vi "Purge uService from local lists.vi"(10 "Last Ack":refnum<class "Last Ack.lvclass">, 11 "Guardian in":refnum<class "Guardian.lvclass">) -> (0 "error out":errorcluster, 1 "uService ID":string, 2 "uService Properties":T1, 3 "Guardian out":refnum<class "Guardian.lvclass">)   [LabVIEW 2020, in "TALOS.lvlib" / "Guardian.lvlib" / "Guardian.lvclass"]
uses:
  Guardian.lvclass
  Guardian.lvclass/Guardian.ctl
  Classes/uService List/uService List.lvclass
  builds/Actor Framework PPL/Actor Framework.lvlibp/1abvi3w/vi.lib/ActorFramework/Message Enqueuer/Message Enqueuer.lvclass
  Classes/uService List/uService Properties.ctl
  TALOS.lvlib
  builds/Actor Framework PPL/Actor Framework.lvlibp/1abvi3w/vi.lib/ActorFramework/LastAck/Last Ack.lvclass
  C:/LabVIEW Code/TALOS/talos/Ancestor/Ancestor/Ancestor.lvclass
  C:/LabVIEW Code/TALOS/builds/Actor Framework PPL/Actor Framework.lvlibp/1abvi3w/vi.lib/ActorFramework/Actor/Actor.lvclass
  C:/LabVIEW Code/TALOS/talos/Guardian/Guardian/Guardian.lvclass
  Classes/Distributed uService Map/Distributed uService Map.lvclass
  Classes/uService List/Get ID from Queue.vi
  Classes/uService List/Remove uService.vi
  Classes/uService List/Get Properties.vi
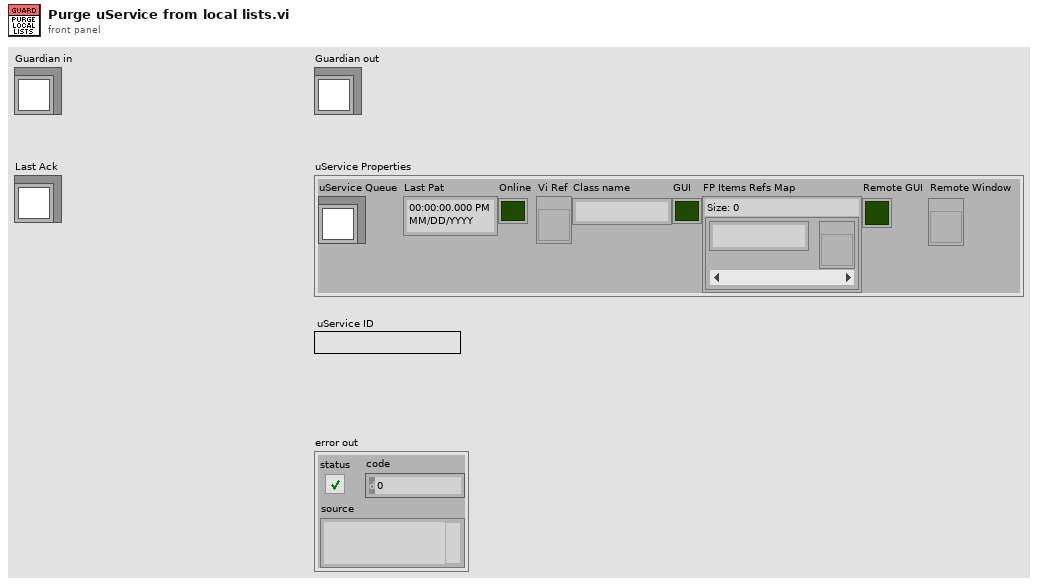
[diagram p1: front panel]
types:
  T1 = typedef "TALOS.lvlib/Classes.lvlib/uService List.lvclass/uService Properties.ctl" = cluster{"uService Queue":refnum<class "Message Enqueuer.lvclass">, "Last Pat":timestamp, "Online":bool, "Vi Ref":refnum<vi>, "Class name":string, "GUI":bool, "FP Items Refs Map":map{string, refnum<vi>}, "Remote GUI":bool, "Remote Window":refnum<vi>}
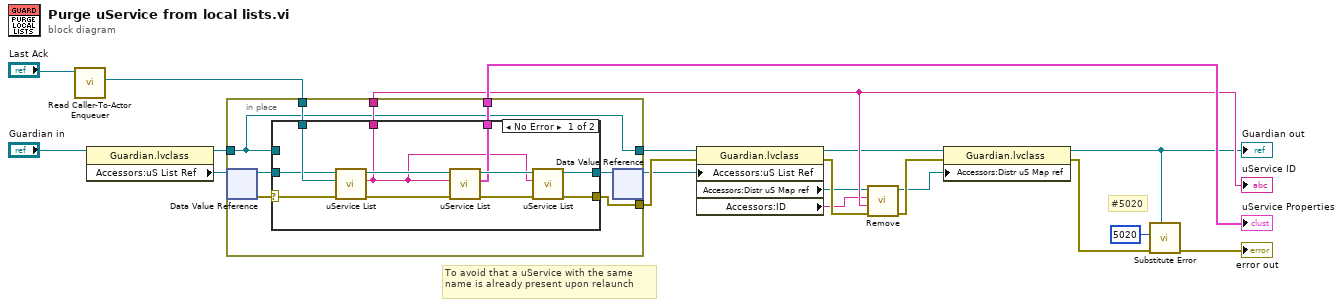
[diagram p0: block diagram]
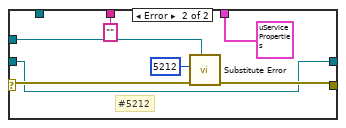
[diagram p2: hidden frame]
diagram:
  # "#5020"
  # "To avoid that a uService with the same name is already present upon relaunch"
  n1 = call "Read Caller-To-Actor Enqueuer.vi"("Last Ack"="Last Ack") -> ("Caller-to-Actor Enqueuer"=w12:refnum<class "Message Enqueuer.lvclass">)  [unwired: 10 in]
  n2 = property class="Guardian.lvclass"(reference="Guardian in") -> (reference out=w16:refnum<class "Guardian.lvclass">, "Accessors:uS List Ref"=w11:refnum<data-value>)  [unwired: 1 in, 1 out]
  n3 = in-place {
    in-place-border: w12 -> [w28]
    in-place-border: [w23] -> w18
    in-place-border: [w26] -> w14
    in-place-border: [w25] -> w19
    in-place-border: w16 -> [w21]
    in-place-border: [w21] -> w17
    n4 = in-place-dvr #1(w11) -> (w27:refnum<class "uService List.lvclass">, w22:errorcluster)
    n5 = case shown="No Error" w22 {
      selector: w22 -> [w29 w45]
      tunnel: w28 -> [w35 _]
      tunnel: w27 -> [w34 w40]
      tunnel: [w33 w43] -> w26
      tunnel: [w32 T1 {"uService Queue"=refnum, "Last Pat"=timestamp(0 s since 1904-01-01), "Online"=FALSE, "Vi Ref"=refnum, "Class name"="", "GUI"=FALSE, "FP Items Refs Map"={}, "Remote GUI"=FALSE, "Remote Window"=refnum} ("uService Properties")] -> w25
      tunnel: [w31 w40] -> w24
      tunnel: [w30 "" ("ID out")] -> w23
      tunnel: w21 -> [_ w44]
      frame No Error {
        n6 = call-poly "uService List.vi"("error in (no error)"=w29, "uService Queue"=w35, "uService List in"=w34) -> ("error out"=w36:errorcluster, "ID out"=w30:string, "uService List out"=w38:refnum<class "uService List.lvclass">)  [unwired: 6 in]
        n7 = call-poly "uService List.vi"("error in (no error)"=w36, "ID"=w30, "uService List in"=w38) -> ("error out"=w37:errorcluster, "uService Properties"=w32:T1, "uService List out"=w39:refnum<class "uService List.lvclass">)  [unwired: 6 in]
        n8 = call-poly "uService List.vi"("error in (no error)"=w37, "ID"=w30, "uService List in"=w39) -> ("error out"=w33:errorcluster, "uService List out"=w31:refnum<class "uService List.lvclass">)  [unwired: 7 in]
      }
      frame Error {
        # "#5212"
        n9 = call "Substitute Error.vi"("LabVIEW Object"=w44, "error in (no error)"=w45, "Error Code"=5212) -> ("error out"=w43:errorcluster)  [unwired: 8 in]
      }
    }
    n10 = in-place-dvr #1(w24) -> (w13:refnum<data-value>)  [unwired: 1 out]
  }
  "uService Properties" <- w19
  "uService ID" <- w18
  n11 = property class="Guardian.lvclass"(reference=w17, error in=w14, "Accessors:uS List Ref"=w13) -> (reference out=w5:refnum<class "Guardian.lvclass">, error out=w20:errorcluster, "Accessors:Distr uS Map ref"=w7:refnum<data-value>, "Accessors:ID"=w6:string)
  n12 = call "Remove.vi"("error in (no error)"=w20, "uService ID"=w18, "Guardian"=w6, "Distr uS Map ref in"=w7) -> ("error out"=w4:errorcluster, "Distr uS Map ref out"=w3:refnum<data-value>)  [unwired: 5 in, 1 out]
  n13 = property class="Guardian.lvclass"(reference=w5, error in=w4, "Accessors:Distr uS Map ref"=w3) -> (reference out=w2:refnum<class "Guardian.lvclass">, error out=w1:errorcluster)
  "Guardian out" <- w2
  n14 = call "Substitute Error.vi"("LabVIEW Object"=w2, "error in (no error)"=w1, "Error Code"=5020) -> ("error out"=→"error out":errorcluster)  [unwired: 8 in]
